vi "wait for.vi"(8 "error in":errorcluster, 11 "Wait Time (ms)":i32) -> (0 "error out":errorcluster)   [LabVIEW 2023, in "Spectrum Analyzer.lvlib"]
uses:
  Spectrum Analyzer.lvlib
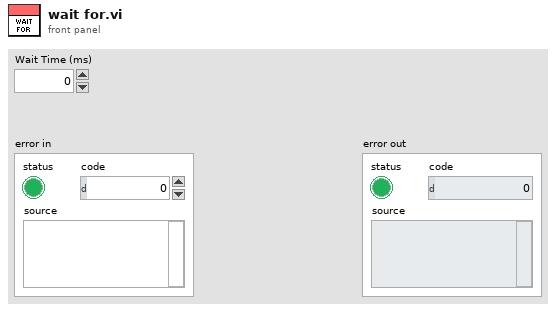
[diagram p1: front panel]
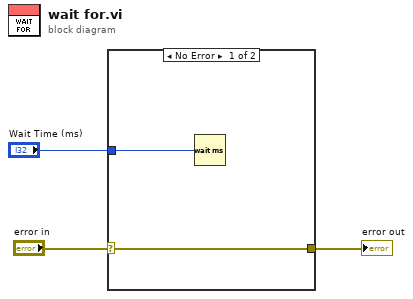
[diagram p0: block diagram]
diagram:
  n1 = case shown="No Error" "error in" {
    selector: "error in" -> [w5 w6]
    tunnel: [w5 w6] -> w2
    tunnel: "Wait Time (ms)" -> [w4 _]
    frame No Error {
      n2 = Wait (ms)(milliseconds to wait=w4) -> ()  [unwired: 1 out]
    }
    frame Error {
    }
  }
  "error out" <- w2
